vi "_script_add_vi_reference_case.vi"(8 "error in (no error)":errorcluster, 9 "Show FP?":bool, 11 "VI Ref":refnum<vi>) -> (0 "error out":errorcluster)   [LabVIEW 2017]
uses:
  _csmHelper/API/Destroy.vi
  _csmHelper/API/Save Instrument.vi
  _csmHelper/API/Stop Undo.vi
  _csmHelper/usecase/Add VI Reference Case.vi
  _csmHelper/API/Start Undo.vi
  _csmHelper/API/Open Front Panel.vi
  _csmHelper/Properties/Read States.vi
  _csmHelper/API/Create From Basic Refs.vi
  _csmHelper/Utility/Is CSM Module - VIRef.vi
  _csmHelper/CSM-Helper.lvclass
  _csmHelper/Utility/CSM-Helper Utility.lvlib
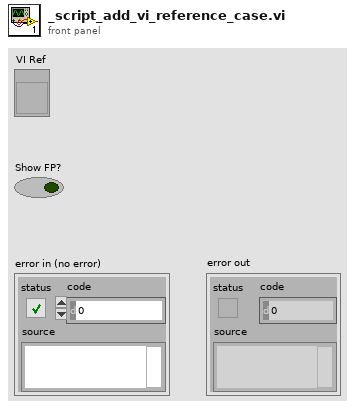
[diagram p1: front panel]
types:
  T1 = typedef "CSM-Helper Utility.lvlib/CSM Basic Refs.ctl" = cluster{"VI":refnum<vi>, "While Loop":refnum<vi>, "Case Structure":refnum<vi>, "Parse State Queue":refnum<vi>, "Event Structure":refnum<vi>, "Type":T2}
  T2 = typedef "CSM-Helper Utility.lvlib/CSM Module Type.ctl" = enum16{"Not a CSM", "JKISM", "CSM"}
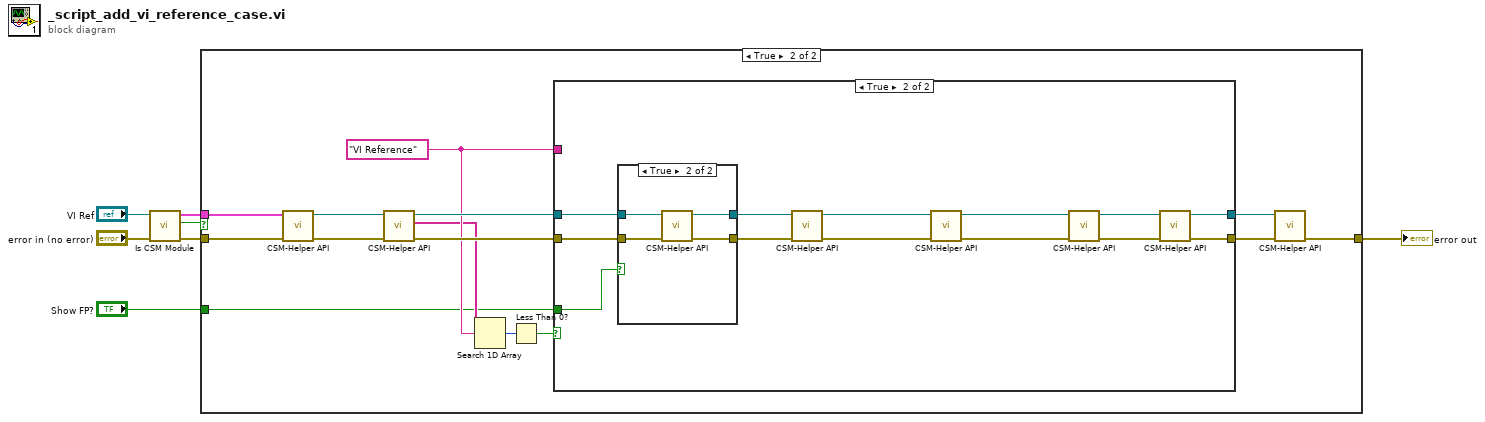
[diagram p0: block diagram]
diagram:
  n1 = call-poly "Is CSM Module.vi"("error in (no error)"="error in (no error)", "VIRef"="VI Ref") -> ("error out"=w4:errorcluster, "Is CSM Module?"=w1:bool, "CSM Basic Refs"=w2:T1)  [unwired: 7 in]
  n2 = case shown="True" w1 {
    tunnel: [w8 w12] -> w6
    tunnel: "Show FP?" -> [_ w11]
    tunnel: w4 -> [w8 w10]
    tunnel: w2 -> [_ w9]
    frame False {
    }
    frame True {
      w16 = "VI Reference" ("element")
      n3 = call-poly "CSM-Helper API.vi"("error in (no error)"=w10, "CSM Basic Refs"=w9) -> ("error out"=w22:errorcluster, "CSM-Helper.lvclass"=w21:refnum<class "CSM-Helper.lvclass">)  [unwired: 8 in]
      n4 = call-poly "CSM-Helper API.vi"("error in (no error)"=w22, "CSM-Helper in"=w21) -> ("error out"=w18:errorcluster, "Value"=w14:string[], "CSM-Helper out"=w19:refnum<class "CSM-Helper.lvclass">)  [unwired: 7 in]
      n5 = Search 1D Array(1D array=w14, element=w16) -> (index of element=w20:i32)  [unwired: 1 in]
      n6 = Less Than 0?(x=w20) -> (x < 0?=w17:bool)
      n7 = case shown="True" w17 {
        tunnel: w19 -> [w23 w37]
        tunnel: w18 -> [w24 w28]
        tunnel: w16 -> [_ _]
        tunnel: [w24 w31] -> w13
        tunnel: [w23 w33] -> w15
        tunnel: w11 -> [_ w27]
        frame False {
        }
        frame True {
          n8 = case shown="True" w27 {
            tunnel: w37 -> [w38 w43]
            tunnel: [w38 w42] -> w30
            tunnel: [w39 w41] -> w29
            tunnel: w28 -> [w39 w40]
            frame False {
            }
            frame True {
              n9 = call-poly "CSM-Helper API.vi"("error in (no error)"=w40, "CSM-Helper in"=w43) -> ("error out"=w41:errorcluster, "CSM-Helper out"=w42:refnum<class "CSM-Helper.lvclass">)  [unwired: 8 in]
            }
          }
          n10 = call-poly "CSM-Helper API.vi"("error in (no error)"=w29, "CSM-Helper in"=w30) -> ("error out"=w35:errorcluster, "CSM-Helper out"=w36:refnum<class "CSM-Helper.lvclass">)  [unwired: 8 in]
          n11 = call-poly "CSM-Helper API.vi"("error in"=w35, "CSM-Helper in"=w36) -> ("error out"=w25:errorcluster, "CSM-Helper out"=w26:refnum<class "CSM-Helper.lvclass">)  [unwired: 8 in]
          n12 = call-poly "CSM-Helper API.vi"("error in (no error)"=w25, "CSM-Helper in"=w26) -> ("error out"=w32:errorcluster, "CSM-Helper out"=w34:refnum<class "CSM-Helper.lvclass">)  [unwired: 8 in]
          n13 = call-poly "CSM-Helper API.vi"("error in (no error)"=w32, "CSM-Helper in"=w34) -> ("error out"=w31:errorcluster, "CSM-Helper out"=w33:refnum<class "CSM-Helper.lvclass">)  [unwired: 8 in]
        }
      }
      n14 = call-poly "CSM-Helper API.vi"("error in (no error)"=w13, "CSM-Helper in"=w15) -> ("error out"=w12:errorcluster)  [unwired: 8 in, 1 out]
    }
  }
  "error out" <- w6
